vi "Scope Tester.vi"() -> ()   [LabVIEW 2018]
uses:
  src/api/logger_class/Failure Information.ctl
  src/api/logger_class/Log Record.ctl
  src/api/logger_class/Internal Log Levels.ctl
  src/api/logger_class/Log Levels.ctl
  src/api/configuration/scopes/basic_scope/Basic.lvclass
  C:/Users/Colin/Documents/software_projects/labview/glog/src/api/extension/scope_interface/Scope.lvclass
  src/api/configuration/handlers/file_handler/File Handler.lvclass
  C:/Users/Colin/Documents/software_projects/labview/glog/src/api/extension/formatting_handler_interface/Formatting Handler.lvclass
  src/api/configuration/scopes/basic_scope/New (Element).vi
  src/api/configuration/handlers/file_handler/New (Single Trigger).vi
  src/api/logger_class/Log (Parts).vi
  src/api/logger_class/Logger.lvclass
  Scope Tester Class.lvclass
  Scope Tester Library.lvlib
panel:
  out "failure info":T1 {"Log Record"."timestamp" format="%<%x %.3X>T"}
  out "error out":errorcluster
  # "Locals"
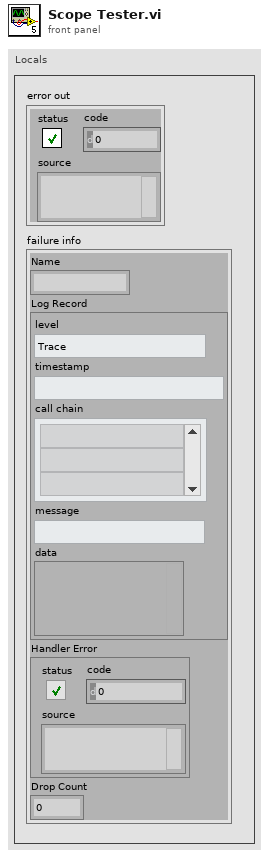
[diagram p1: front panel]
types:
  T1 = typedef "GLog.lvlib/Logger.lvclass/Failure Information.ctl" = cluster{"Name":string, "Log Record":T2, "Handler Error":errorcluster, "Drop Count":u32}
  T2 = typedef "GLog.lvlib/Logger.lvclass/Log Record.ctl" = cluster{"level":T3, "timestamp":timestamp, "call chain":string[], "message":string, "data":variant}
  T3 = typedef "GLog.lvlib/Logger.lvclass/Internal Log Levels.ctl" = enum16{"Trace", "Debug", "Info", "Warning", "Error", "Critical", "Internal"}
  T4 = typedef "GLog.lvlib/Logger.lvclass/Log Levels.ctl" = enum16{"Trace", "Debug", "Info", "Warning", "Error", "Critical"}
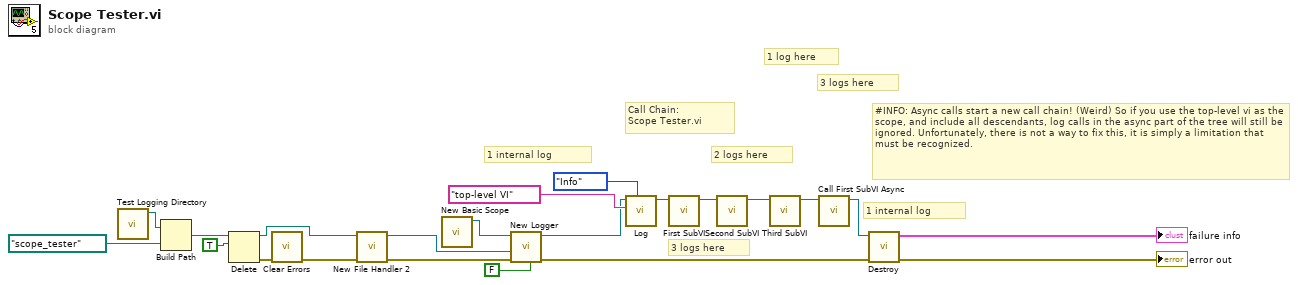
[diagram p0: block diagram]
diagram:
  # "#INFO: Async calls start a new call chain! (Weird) So if you use the top-level vi as the scope, and include all descendants, log calls in the async part of the tree will still be ignored. Unfortunately, there is not a way to fix this, it is simply a limitation that must be recognized."
  # "3 logs here"
  # "1 log here"
  # "2 logs here"
  # "1 internal log"
  # "3 logs here"
  # "Call Chain:\nScope Tester.vi"
  # "1 internal log"
  n1 = call "Test Logging Directory.vi"() -> ("test logging directory"=w6:path)  [unwired: 11 in]
  n2 = Build Path(base path=w6, name or relative path=path "scope_tester" ("base path")) -> (appended path=w5:path)
  n3 = Delete(path (use dialog)=w5, entire hierarchy (F)=TRUE) -> (deleted path=w4:path, error out=w8:errorcluster)  [unwired: 3 in, 1 out]
  n4 = call <vilib>:"Clear Errors.vi"("error in (no error)"=w8) -> ("error out"=w2:errorcluster)  [unwired: 5 in, 1 out]
  n5 = call-poly "New File Handler 2.vi"("error in"=w2, "log directory (<app dir>/logs)"=w4) -> ("error out"=w1:errorcluster, "file handler"=w3:refnum<class "File Handler.lvclass">)  [unwired: 7 in, 1 out]
  n6 = call-poly "New Basic Scope.vi"() -> ("basic scope"=w22:refnum<class "Basic.lvclass">)  [unwired: 11 in]
  n7 = call "New Logger.vi"("dialog on failure? (T)"=FALSE, "error in (no error)"=w1, "log handler (file handler)"=w3, "logger scope (all)"=w22) -> ("error out"=w16:errorcluster, "logger"=w20:refnum<class "Logger.lvclass">)  [unwired: 6 in]
  n8 = call-poly "Log.vi"("log level"=Log_Levels."Info" ("level"), "message"="top-level VI", "logger in"=w20) -> ("logger out"=w18:refnum<class "Logger.lvclass">)  [unwired: 8 in]
  n9 = call "First SubVI.vi"("logger in"=w18) -> ("logger out"=w12:refnum<class "Logger.lvclass">)  [unwired: 10 in]
  n10 = call "Second SubVI.vi"("logger in"=w12) -> ("logger out"=w11:refnum<class "Logger.lvclass">)  [unwired: 10 in]
  n11 = call "Third SubVI.vi"("logger in"=w11) -> ("logger out"=w10:refnum<class "Logger.lvclass">)  [unwired: 10 in]
  n12 = call "Call First SubVI Async.vi"("logger in"=w10) -> ("logger out"=w9:refnum<class "Logger.lvclass">)  [unwired: 10 in]
  n13 = call "Destroy.vi"("error in (no error)"=w16, "logger in"=w9) -> ("error out"=→"error out":errorcluster, "failure info"=→"failure info":T1)  [unwired: 8 in]
